vi "VIH Utility - UI - Display Formatted Text (String Control).vi"(8 "error in":errorcluster, 10 "Formatted text":string, 11 "Str Refnum":refnum<vi>) -> (0 "error out":errorcluster, 3 "dup Str Refnum":refnum<vi>)   [LabVIEW 2014]
doc: "::: VI Helpeks :::\nCopyright (c) 2000-2026 Konstantin Shifershteyn. All rights reserved."
panel:
  # "VI Helpeks\nCopyright (c) 2012-2026 Konstantin Shifershteyn"
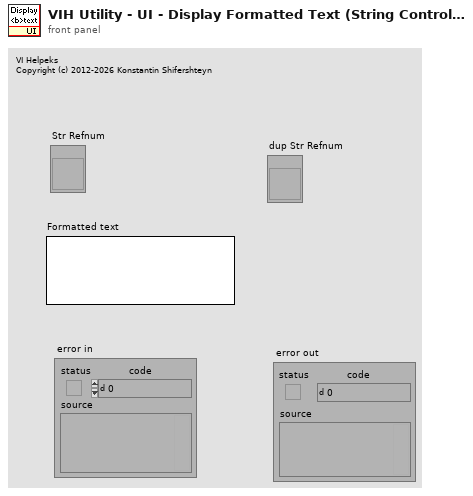
[diagram p1: front panel]
types:
  T1 = cluster{"Selection Start":u32, "Selection End":i32}
  T2 = cluster{"tag":string, "Start":i32, "Start":i32}[]
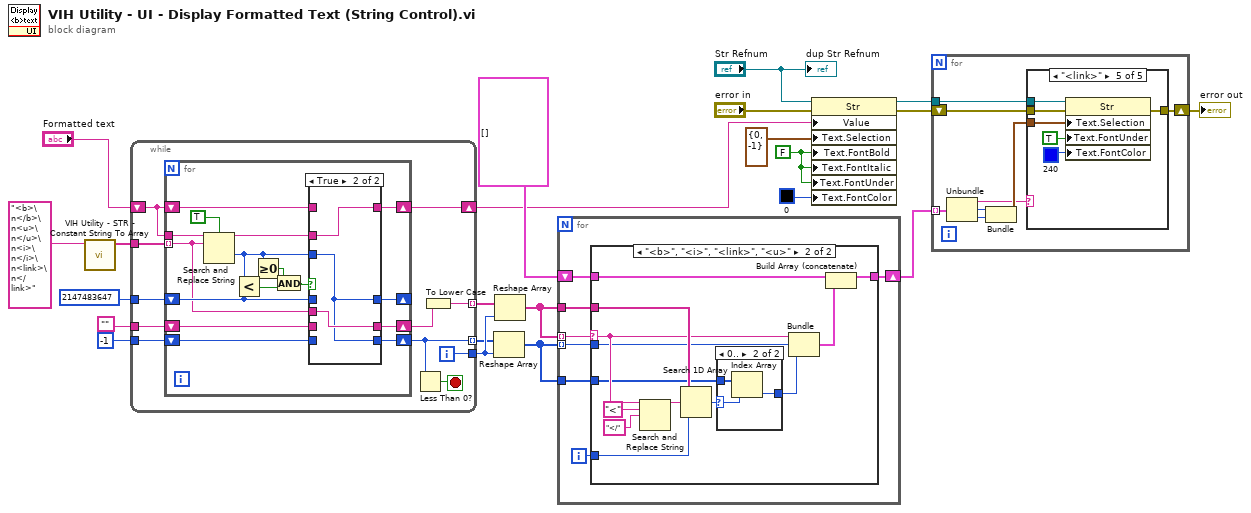
[diagram p0: block diagram]
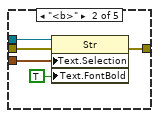
[diagram p3: hidden frame]
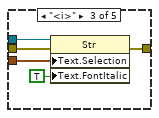
[diagram p4: hidden frame]
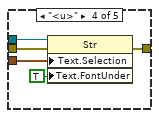
[diagram p5: hidden frame]
diagram:
  w15 = FALSE
  n1 = call "VIH Utility - STR - Constant String To Array.vi"("String in"="<b>\n</b>\n<u>\n</u>\n<i>\n</i>\n<link>\n</link>") -> ("Array out"=w7:string[])  [unwired: 10 in]
  n2 = while {
    tunnel: w7 -> [w33]
    shift-right: [w31] -> w14
    shift-left: "Formatted text" -> [w32]
    tunnel: [w27] -> w8 mode=indexing
    tunnel: [w29] -> w10
    tunnel: [w28] -> w9 mode=indexing
    tunnel: 2147483647 -> [w25]
    tunnel: "" -> [w24]
    tunnel: -1 ("Start") -> [w23]
    i -> [w29]
    stop <- w30 stop-if-true
    n3 = for {
      tunnel: w32 -> [w49]
      tunnel: w33 -> [w42] mode=indexing
      shift-right: [w47] -> _
      shift-left: w25 -> [w46]
      shift-right: [w45] -> w31
      shift-left: w32 -> [w44]
      shift-right: [w41] -> w27
      shift-left: w23 -> [w40]
      shift-right: [w35] -> w26
      shift-left: w24 -> [w34]
      n4 = Search and Replace String(case sensitive?=TRUE, input string=w49, search string=w42) -> (result string=w43:string, offset past replacement=w38:i32)  [unwired: 5 in, 2 out]
      n5 = Less?(x=w38, y=w46) -> (x < y?=w39:bool)
      n6 = Greater Or Equal To 0?(x=w38) -> (x >= 0?=w37:bool)
      n7 = And(x=w37, y=w39) -> (x .and. y?=w36:bool)
      n8 = case shown="True" w36 {
        tunnel: [w53 w54] -> w47
        tunnel: w38 -> [_ w54]
        tunnel: w46 -> [w53 _]
        tunnel: [w52 w56] -> w45
        tunnel: w44 -> [w52 _]
        tunnel: w43 -> [_ w56]
        tunnel: w42 -> [_ w55]
        tunnel: [w51 w54] -> w41
        tunnel: w40 -> [w51 _]
        tunnel: [w50 w55] -> w35
        tunnel: w34 -> [w50 _]
        frame False {
        }
        frame True {
        }
      }
    }
    n9 = Less Than 0?(x=w27) -> (x < 0?=w30:bool)
    n10 = To Lower Case(string=w26) -> (all lower case string=w28:string)
  }
  n11 = Reshape Array(w8, w10) -> (w21:i32[])
  n12 = Reshape Array(w9, w10) -> (w20:string[])
  n13 = for {
    tunnel: w21 -> [w58] mode=indexing
    tunnel: w20 -> [w63]
    shift-right: [w61] -> w22
    shift-left: cluster{"tag":string, "Start":i32, "End":i32}[] [] -> [w60]
    tunnel: w20 -> [w59] mode=indexing
    tunnel: w21 -> [w57]
    i -> [w62]
    n14 = case shown="\"<b>\", \"<i>\", \"<link>\", \"<u>\"" w59 {
      selector: w59 -> [_ w74]
      tunnel: w63 -> [_ w77]
      tunnel: w62 -> [_ w76]
      tunnel: [w64 w66] -> w61
      tunnel: w60 -> [w64 w67]
      tunnel: w58 -> [_ w70]
      tunnel: w57 -> [_ w69]
      frame Default {
      }
      frame "<b>", "<i>", "<link>", "<u>" {
        n15 = Search and Replace String(input string=w74, search string="<", replace string="</" ("search string")) -> (result string=w71:string)  [unwired: 5 in, 3 out]
        n16 = Search 1D Array(1D array=w77, element=w71, start index (0)=w76) -> (index of element=w75:i32)
        n17 = case shown="0.." w75 {
          selector: w75 -> [w78 w81]
          tunnel: w69 -> [_ w80]
          tunnel: [w78 w79] -> w68
          frame ..-1 {
          }
          frame 0.. {
            n18 = Index Array(array=w80, index=w81) -> (element=w79:i32)
          }
        }
        n19 = Bundle(w74, "Start"=w70, "Start"=w68) -> (w65:cluster{string, "Start":i32, "Start":i32})  [unwired: 1 in]
        n20 = Build Array (concatenate)(w67, w65) -> (w66:T2)
      }
    }
  }
  n21 = property class="Str"(reference="Str Refnum", error in="error in", "Value"=w14, "Text.Selection"=T1 {"Selection Start"=0, "Selection End"=-1}, "Text.FontBold"=w15, "Text.FontItalic"=w15, "Text.FontUnder"=w15, "Text.FontColor"=u32 0) -> (reference out=w11:refnum<vi>, error out=w13:errorcluster)
  n22 = for {
    tunnel: w11 -> [w89]
    shift-right: [w87] -> w5
    shift-left: w13 -> [w88]
    tunnel: w22 -> [w86] mode=indexing
    n23 = Unbundle(w86) -> ("tag"=w82:string, "Start"=w85:i32, "End"=w84:i32)
    n24 = Bundle("Start"=w85, "End"=w84) -> (w83:cluster{"Start":i32, "End":i32})  [unwired: 1 in]
    n25 = case shown="\"<link>\"" w82 {
      tunnel: w89 -> [_ w95 w100 w105 w111]
      tunnel: w88 -> [w90 w93 w98 w103 w109]
      tunnel: [w90 w92 w97 w102 w108] -> w87
      tunnel: w83 -> [_ w91 w96 w101 w107]
      frame Default {
      }
      frame "<b>" {
        n26 = property class="Str"(reference=w95, error in=w93, "Text.Selection"=w91, "Text.FontBold"=TRUE) -> (error out=w92:errorcluster)  [unwired: 1 out]
      }
      frame "<i>" {
        n27 = property class="Str"(reference=w100, error in=w98, "Text.Selection"=w96, "Text.FontItalic"=TRUE) -> (error out=w97:errorcluster)  [unwired: 1 out]
      }
      frame "<u>" {
        n28 = property class="Str"(reference=w105, error in=w103, "Text.Selection"=w101, "Text.FontUnder"=TRUE) -> (error out=w102:errorcluster)  [unwired: 1 out]
      }
      frame "<link>" {
        n29 = property class="Str"(reference=w111, error in=w109, "Text.Selection"=w107, "Text.FontUnder"=TRUE, "Text.FontColor"=u32 240) -> (error out=w108:errorcluster)  [unwired: 1 out]
      }
    }
  }
  "error out" <- w5
  "dup Str Refnum" <- "Str Refnum"
